vi "update 2D array.vi"(7 "Interpret as Unicode (T)":bool, 8 "error in (no error)":errorcluster, 10 "Value":string[][](array[string]), 11 "String Array (2D) Ref":refnum<vi>) -> (0 "error out":errorcluster, 3 "String Array (2D) Ref":refnum<vi>)   [LabVIEW 2019, in "Language Selection.lvlib"]
doc: "Uses \"Value\" input array to translate a 2D array control.\n- - -\nCopyright (c) 2026, Merecs Engineering GmbH"
uses:
  Language Selection.lvlib
panel:
  # "Connector Pane"
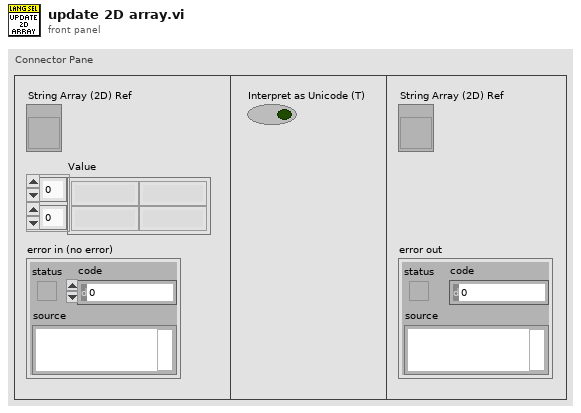
[diagram p1: front panel]
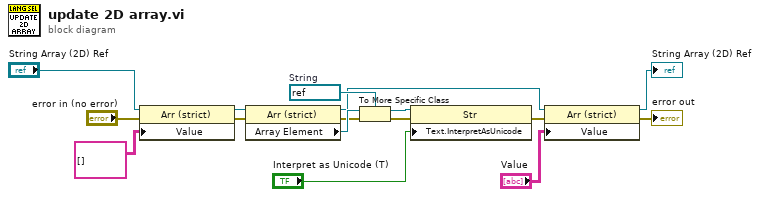
[diagram p0: block diagram]
diagram:
  w14 = refnum<vi> refnum  # String
  n1 = property class="Arr (strict)"(reference="String Array (2D) Ref", error in="error in (no error)", "Value"=string[][] []) -> (reference out=w9:refnum<vi>, error out=w8:errorcluster)
  n2 = property class="Arr (strict)"(reference=w9, error in=w8) -> (reference out=w10:refnum<vi>, error out=w13:errorcluster, "Array Element"=w16:refnum<vi>)
  n3 = To More Specific Class(target class=w14, reference=w16, error in=w13) -> (specific class reference=w15:refnum<vi>, error out=w12:errorcluster)
  n4 = property class="Str"(reference=w15, error in=w12, "Text.InterpretAsUnicode"="Interpret as Unicode (T)") -> (error out=w11:errorcluster)  [unwired: 1 out]
  n5 = property class="Arr (strict)"(reference=w10, error in=w11, "Value"="Value") -> (reference out=→"String Array (2D) Ref":refnum<vi>, error out=→"error out":errorcluster)
